vi "Create VI Overview Picture.vi"(10 "VI Name":string, 11 "Selected CTRLs":T3[](array[typedef])) -> (1 "image size":T2, 2 "Origin":T1, 3 "2D Picture":picture)   [LabVIEW 2019, in "Language Editor.lvlib"]
doc: "- - -\nCopyright (c) 2026, Merecs Engineering GmbH"
uses:
  Language Editor.lvlib
  type defs/Cluster VI controls.ctl
  <vilib>/Utility/miscctls.llb/LVBoundsTypeDef.ctl
  <vilib>/Utility/miscctls.llb/LVPointTypeDef.ctl
panel:
  # "Connector Pane"
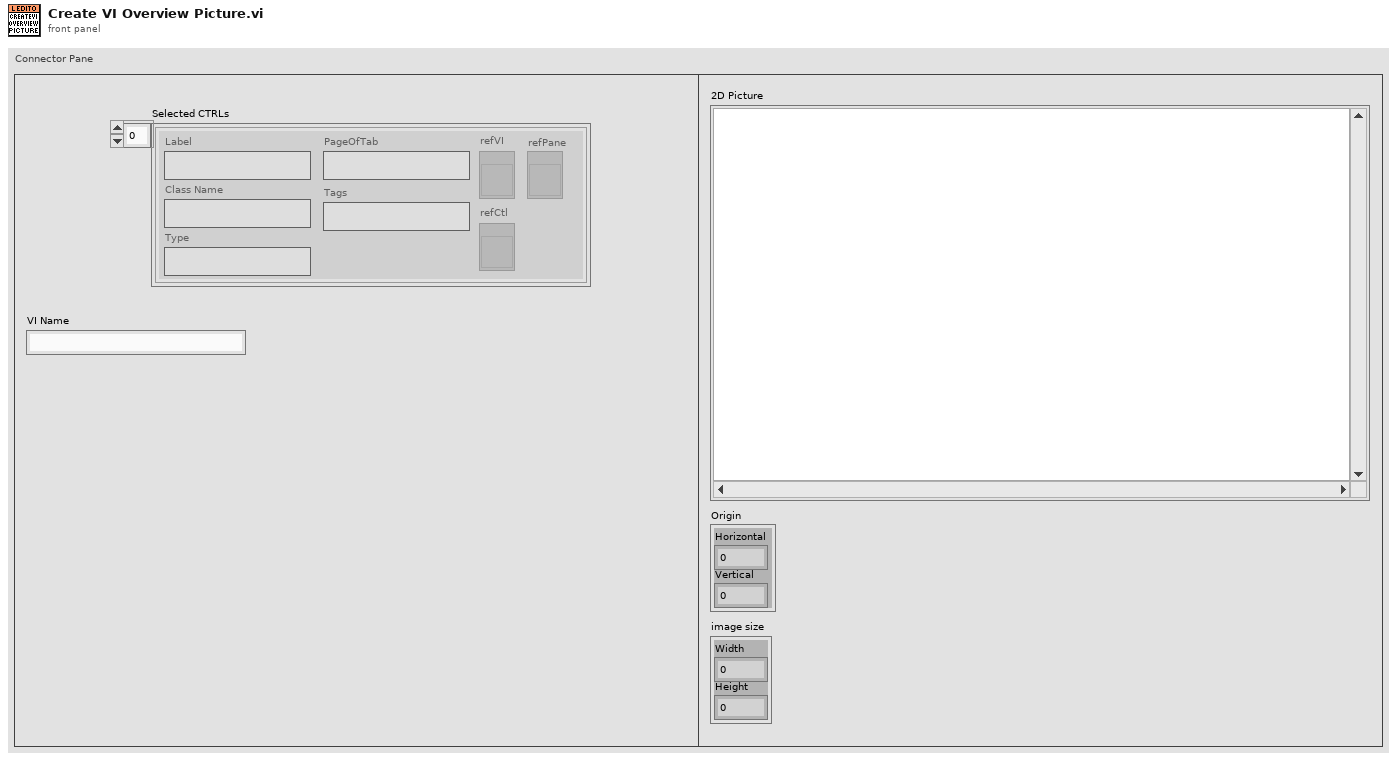
[diagram p1: front panel]
types:
  T1 = typedef "LVPointTypeDef.ctl" = cluster{"Horizontal":i16, "Vertical":i16}
  T2 = typedef "LVBoundsTypeDef.ctl" = cluster{"Width":u32, "Height":u32}
  T3 = typedef "Language Editor.lvlib/Cluster VI controls.ctl" = cluster{"Label":string, "Class Name":string, "Type":string, "Tags":string, "refVI":refnum<vi>, "refCtl":refnum<vi>, "PageOfTab":string, "refPane":refnum<vi>}
  T4 = cluster{"Horizintal":i32, "Right":i32, "Vertical":i32, "Bottom":i32}
  T5 = cluster{"Width":u16, "Style":enum32{"Solid", "Dash", "Dot", "DashDot", "DashDotDot"}}
  T6 = cluster{"left":i16, "top":i16, "right":i16, "bottom":i16}
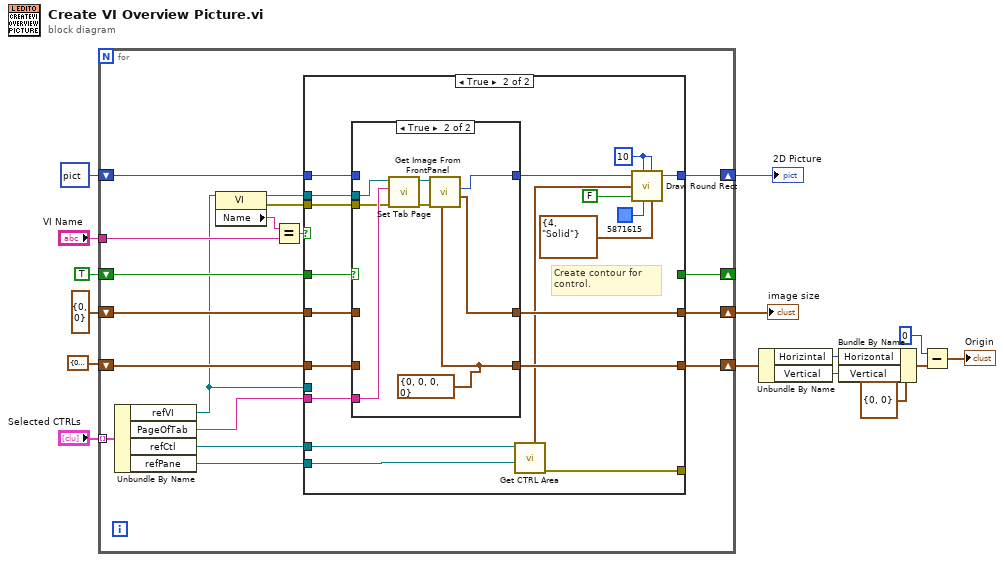
[diagram p0: block diagram]
diagram:
  n1 = for {
    tunnel: "Selected CTRLs" -> [w33] mode=indexing
    tunnel: "VI Name" -> [w32]
    shift-right: [w28] -> w12
    shift-left: picture data[5B] ("new picture") -> [w27]
    shift-right: [w26] -> _
    shift-left: TRUE -> [w25]
    shift-right: [w22] -> w10
    shift-left: T2 {"Width"=0, "Height"=0} ("output cluster") -> [w21]
    shift-right: [w20] -> w2
    shift-left: T4 {"Horizintal"=0, "Right"=0, "Vertical"=0, "Bottom"=0} ("Bounds") -> [w19]
    n2 = Unbundle By Name(w33) -> ("refVI"=w18:refnum<vi>, "PageOfTab"=w24:string, "refCtl"=w16:refnum<vi>, "refPane"=w17:refnum<vi>)
    n3 = property class="VI"(reference=w18) -> (reference out=w29:refnum<vi>, error out=w23:errorcluster, "Name"=w31:string)  [unwired: 1 in]
    n4 = Equal?(x=w31, y=w32) -> (x = y?=w30:bool)
    n5 = case shown="True" w30 {
      tunnel: w16 -> [_ w40]
      tunnel: w29 -> [_ w46]
      tunnel: [w37 w53] -> w28
      tunnel: w27 -> [w37 w51]
      tunnel: [w36 _] -> w26
      tunnel: w25 -> [w36 w49]
      tunnel: w24 -> [_ w48]
      tunnel: w23 -> [_ w47]
      tunnel: [w35 w45] -> w22
      tunnel: w21 -> [w35 w44]
      tunnel: [w34 w43] -> w20
      tunnel: w19 -> [w34 w42]
      tunnel: w18 -> [_ _]
      tunnel: w17 -> [_ w39]
      tunnel: [_ w38] -> _
      frame False {
      }
      frame True {
        w56 = i16 10 ("oval width")
        # "Create contour for control."
        n6 = case shown="True" w49 {
          tunnel: w46 -> [_ w66]
          tunnel: w51 -> [w59 _]
          tunnel: [w59 w62] -> w50
          tunnel: w48 -> [_ w67]
          tunnel: w47 -> [_ w65]
          tunnel: [w58 w61] -> w45
          tunnel: w44 -> [w58 _]
          tunnel: [w57 w60] -> w43
          tunnel: w42 -> [w57 _]
          frame False {
          }
          frame True {
            w60 = T4 {"Horizintal"=0, "Right"=0, "Vertical"=0, "Bottom"=0} ("Bounds")
            n7 = call "Set Tab Page.vi"("error in (no error)"=w65, "PageOfTab"=w67, "VI in"=w66) -> ("error out"=w63:errorcluster, "VI out"=w64:refnum<vi>)  [unwired: 7 in]
            n8 = call "Get Image From FrontPanel.vi"("Bounds"=w60, "error in (no error)"=w63, "vi reference"=w64) -> ("image size"=w61:T2, "image"=w62:picture)  [unwired: 5 in, 2 out]
          }
        }
        n9 = call "Get CTRL Area.vi"("Pane in"=w39, "Control in"=w40) -> ("error out"=w38:errorcluster, "CTRL Area"=w41:T6)  [unwired: 5 in, 3 out]
        n10 = call <vilib>:"Draw Round Rect.vi"("picture"=w50, "oval width"=w56, "rect"=w41, "fill?(F)"=FALSE, "color(black)"=u32 5871615, "oval height"=w56, "pen"=T5 {"Width"=4, "Style"=enum."Solid"}) -> ("new picture"=w53:picture)  [unwired: 2 in]
      }
    }
  }
  "2D Picture" <- w12
  "image size" <- w10
  n11 = Unbundle By Name(w2) -> ("Horizintal"=w6:i32, "Vertical"=w7:i32)
  n12 = Bundle By Name(cluster=T1 {"Horizontal"=0, "Vertical"=0} ("Origin"), "Horizontal"=w6, "Vertical"=w7) -> (w5:T1)
  n13 = Subtract(x=u32 0 ("upper limit"), y=w5) -> (x-y=→"Origin":cluster{"Horizontal":u32, "Vertical":u32})
